vi "post semaphores.vi"(8 "error in (no error)":errorcluster, 11 "semaphores in":T1[](array[typedef])) -> (0 "error out":errorcluster, 3 "semaphores out":T1[](array[typedef]))   [LabVIEW 2014, in "Shared Memory runtime.lvclass"]
uses:
  Shared Memory runtime.lvclass
  controls/semaphore data.ctl
  <vilib>/NI/NI Linux RT IPC/POSIX Threads/Classes/Semaphore/Controls/reference.ctl
  <vilib>/NI/NI Linux RT IPC/POSIX Threads/Classes/Semaphore/Semaphore.lvclass
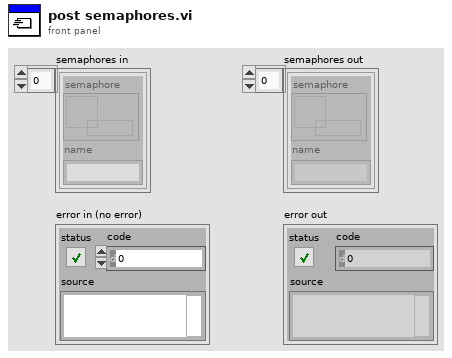
[diagram p1: front panel]
types:
  T1 = typedef "Shared Memory runtime.lvclass/semaphore data.ctl" = cluster{"semaphore":T2, "name":string}
  T2 = typedef "Linux RT IPC.POSIX Threads.lvlib/Semaphore.lvclass/reference.ctl" = refnum<data-value>
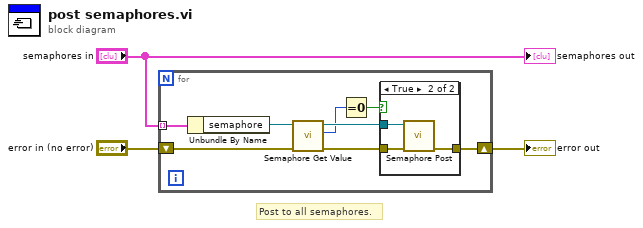
[diagram p0: block diagram]
diagram:
  # "Post to all semaphores."
  n1 = for {
    shift-right: [w10] -> w2
    shift-left: "error in (no error)" -> [w11]
    tunnel: "semaphores in" -> [w9] mode=indexing
    n2 = Unbundle By Name(w9) -> ("semaphore"=w7:T2)
    n3 = call <vilib>:"Semaphore Get Value.vi"("error in (no error)"=w11, "Semaphore in"=w7) -> ("error out"=w8:errorcluster, "value"=w5:i32, "Semaphore out"=w6:T2)  [unwired: 7 in]
    n4 = Equal To 0?(x=w5) -> (x = 0?=w4:bool)
    n5 = case shown="True" w4 {
      tunnel: w8 -> [w12 w15]
      tunnel: [w12 w14] -> w10
      tunnel: w6 -> [_ w13]
      frame False {
      }
      frame True {
        n6 = call <vilib>:"Semaphore Post.vi"("error in (no error)"=w15, "Semaphore in"=w13) -> ("error out"=w14:errorcluster)  [unwired: 8 in, 1 out]
      }
    }
  }
  "error out" <- w2
  "semaphores out" <- "semaphores in"
